vi "refresh table.vi"(5 "channels ref":refnum<vi>, 7 "Mappings":refnum<vi>, 8 "error in":errorcluster, 10 "Modules Configurations":refnum<class "TBM module configuration.lvclass">[](array[class]), 11 "engine configuration in":refnum<class "engine configuration.lvclass">) -> (0 "error out":errorcluster)   [LabVIEW 2013, in "PL Framework Configuration Tool.lvlib" / "Engine Mappings.lvclass"]
uses:
  Engine Mappings.lvclass
  <vilib>/NI/Module Execution Interface/Engine Configuration/engine configuration.lvclass
  <vilib>/NI/Tag Bus Module Framework/module configuration/TBM module configuration.lvclass
  <vilib>/NI/Tag Bus Module Framework/channel/TBM channel.lvclass/TBM channel.ctl
  <vilib>/NI/Tag Bus/tag/tag descriptor.lvclass/tag descriptor.ctl
  <vilib>/NI/Tag Bus/tag/tag descriptor.lvclass
  <vilib>/NI/Tag Bus Module Framework/channel/TBM channel.lvclass
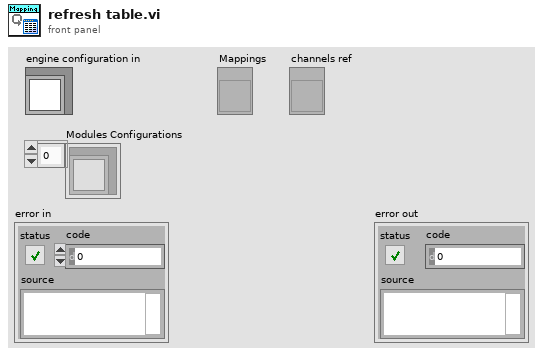
[diagram p1: front panel]
types:
  T1 = typedef "PL Framework Configuration Tool.lvlib/Engine Mappings.lvclass/module information.ctl" = cluster{"display name":string, "instance id":string, "channels":refnum<class "TBM channel.lvclass">[]}
  T2 = typedef "TBM channel.lvclass/channel classification.ctl" = enum16{"input data", "output data", "processing parameter", "processing result"}
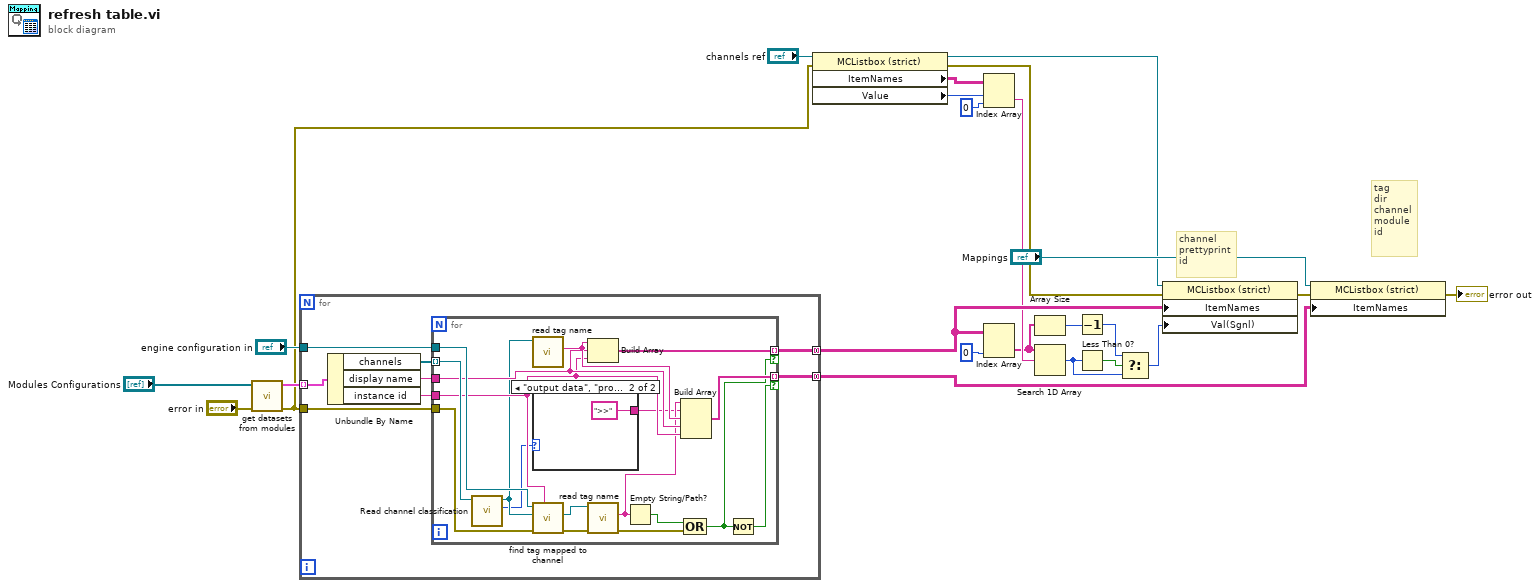
[diagram p0: block diagram]
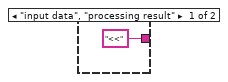
[diagram p2: hidden frame]
diagram:
  # "channel\nprettyprint\nid"
  # "tag\ndir\nchannel\nmodule\nid"
  n1 = call "get datasets from modules.vi"("error in"="error in", "Modules Configurations"="Modules Configurations") -> ("error out"=w16:errorcluster, "module datasets"=w17:T1[])  [unwired: 8 in]
  n2 = for {
    tunnel: w17 -> [w32] mode=indexing
    tunnel: w16 -> [w28]
    tunnel: "engine configuration in" -> [w27]
    tunnel: [w26] -> w9 mode=concatenating
    tunnel: [w25] -> w19 mode=concatenating
    n3 = Unbundle By Name(w32) -> ("channels"=w31:refnum<class "TBM channel.lvclass">[], "display name"=w30:string, "instance id"=w29:string)
    n4 = for {
      tunnel: w31 -> [w48] mode=indexing
      tunnel: w30 -> [w42]
      tunnel: w29 -> [w41]
      tunnel: w28 -> [w49]
      tunnel: w27 -> [w50]
      tunnel: [w45] -> w26 mode=indexing if=w37
      tunnel: [w44] -> w25 mode=indexing if=w36
      n5 = call <vilib>:"Read channel classification.vi"("channel in"=w48) -> ("channel classification"=w34:T2, "channel out"=w35:refnum<class "TBM channel.lvclass">)  [unwired: 8 in, 1 out]
      n6 = call <vilib>:"read tag name.vi"("system tag in"=w35) -> ("name"=w43:string)  [unwired: 8 in, 2 out]
      n7 = case shown="\"output data\", \"processing parameter\"" w34 {
        tunnel: ["<<" ">>"] -> w33
        frame "input data", "processing result" {
        }
        frame "output data", "processing parameter" {
        }
      }
      n8 = call <vilib>:"find tag mapped to channel.vi"("owner"=w41, "error in"=w49, "channel"=w35, "engine configuration in"=w50) -> ("error out"=w47:errorcluster, "tag"=w46:refnum<class "tag descriptor.lvclass">)  [unwired: 5 in, 1 out]
      n9 = Build Array(w43, w42, w41) -> (w45:string[])
      n10 = call <vilib>:"read tag name.vi"("error in"=w47, "system tag in"=w46) -> ("error out"=w38:errorcluster, "name"=w40:string)  [unwired: 7 in, 1 out]
      n11 = Empty String/Path?(string/path=w40) -> (empty?=w39:bool)
      n12 = Build Array(w40, w33, w43, w42, w41) -> (w44:string[])
      n13 = Compound Arithmetic op=OR(w39, w38) -> (w37:bool)
      n14 = Not(x=w37) -> (.not. x?=w36:bool)
    }
  }
  n15 = property class="MCListbox (strict)"(reference="channels ref", error in=w16) -> (reference out=w13:refnum<vi>, error out=w15:errorcluster, "ItemNames"=w12:string[][], "Value"=w8:i32)
  n16 = Index Array(array=w12, index (row)=w8, index (col)=0 ("disabled index (col)")) -> (element=w7:string)
  n17 = Index Array(array=w9, index (col)=0 ("disabled index (col)")) -> (element=w3:string[])  [unwired: 1 in]
  n18 = Array Size(array=w3) -> (size(s)=w2:i32)
  n19 = Search 1D Array(1D array=w3, element=w7) -> (index of element=w5:i32)  [unwired: 1 in]
  n20 = Decrement(x=w2) -> (x-1=w1:i32)
  n21 = Less Than 0?(x=w5) -> (x < 0?=w6:bool)
  n22 = Select(t=w1, s=w6, f=w5) -> (s? t:f=w4:i32)
  n23 = property class="MCListbox (strict)"(reference=w13, error in=w15, "ItemNames"=w9, "Val(Sgnl)"=w4) -> (error out=w22:errorcluster)  [unwired: 1 out]
  n24 = property class="MCListbox (strict)"(reference="Mappings", error in=w22, "ItemNames"=w19) -> (error out=→"error out":errorcluster)  [unwired: 1 out]
